vi "GDSIconEditor_HeaderEditorDialog.vi"(0 "NoSplitter":bool, 1 "BodyBackGround":u32(colorbox), 2 "HeaderText":string, 5 "error in (no error)":errorcluster, 6 "HeaderIconIn":u8[][](array[numeric]) format="%x", 7 "Type":T2, 8 "FrameThickness(1)":u32=1, 9 "ClassBodyIcon":string, 10 "FrameColor":u32(colorbox)) -> (14 "NoSplitterOut":bool, 15 "Cancelled":bool, 16 "FrameColorOut":u32(colorbox), 17 "FrameThicknessOut":u32=1, 18 "HeaderIconOut":u8[][](array[numeric]) format="%x", 19 "error out":errorcluster)   [LabVIEW 2020]
uses:
  <resource>/Framework/Providers/Open_GDS/ClassProviders/Common/LvIcon_class/GDSLvIcon_ColorControl.ctl
  <resource>/Framework/Providers/Open_GDS/ClassProviders/Common/LvIcon_class/GDSLvIcon_Type.ctl
  <vilib>/Utility/miscctls.llb/LVPoint32TypeDef.ctl
  <resource>/Framework/Providers/Open_GDS/ClassProviders/Common/LvIcon_class/GDSLvIcon_ClassColorTypes.ctl
  <resource>/Framework/Providers/Open_GDS/ClassProviders/Common/LvIcon_class/subvis/GDSLvIcon_TextDataType.ctl
  <resource>/Framework/Providers/Open_GDS/ClassProviders/Common/LvIcon_class/GDSLvIcon_WordCompressionType.ctl
  <resource>/Framework/Providers/Open_GDS/ClassProviders/Common/LvIcon_class/GDSLvIcon_TextAlignment.ctl
  <vilib>/event_ctls.llb/lveventtype.ctl
  <vilib>/Analysis/NI_AALBase.lvlib
panel:
  out "Coords 2":T1
  out "Coords":T1
  in  "_LastHeaders":picture[](array[picture]) caption="Last used headers"
  in  "Help":bool
  in  "Dice":cluster{"Boolean 2":bool, "Dice 2":bool}
  out "Icon Preview":picture
  in  "Frame":T3 caption="Color"
  in  "Thickness (pixels)":u8=3 min=1 max=3 step=1
  in  "Rows":enum16{"1 Row", "2 Rows", "3 Rows"}(ring)
  in  "Font Compression":enum16{"Auto", "On", "Off"}(ring)
  in  "CapitalOnly":bool=TRUE caption="Only use capital characters"
  in  "Height (pixels)":u8=9 min=5 max=19
  in  "Text":string="Endevo"
  in  "HeaderBk":T3 caption="Background"
  in  "HeaderText":T3 caption="Text"
  in  "OK":bool
  in  "Cancel":bool
  # "Header"
  # "Random color generation"
  # "Frame"
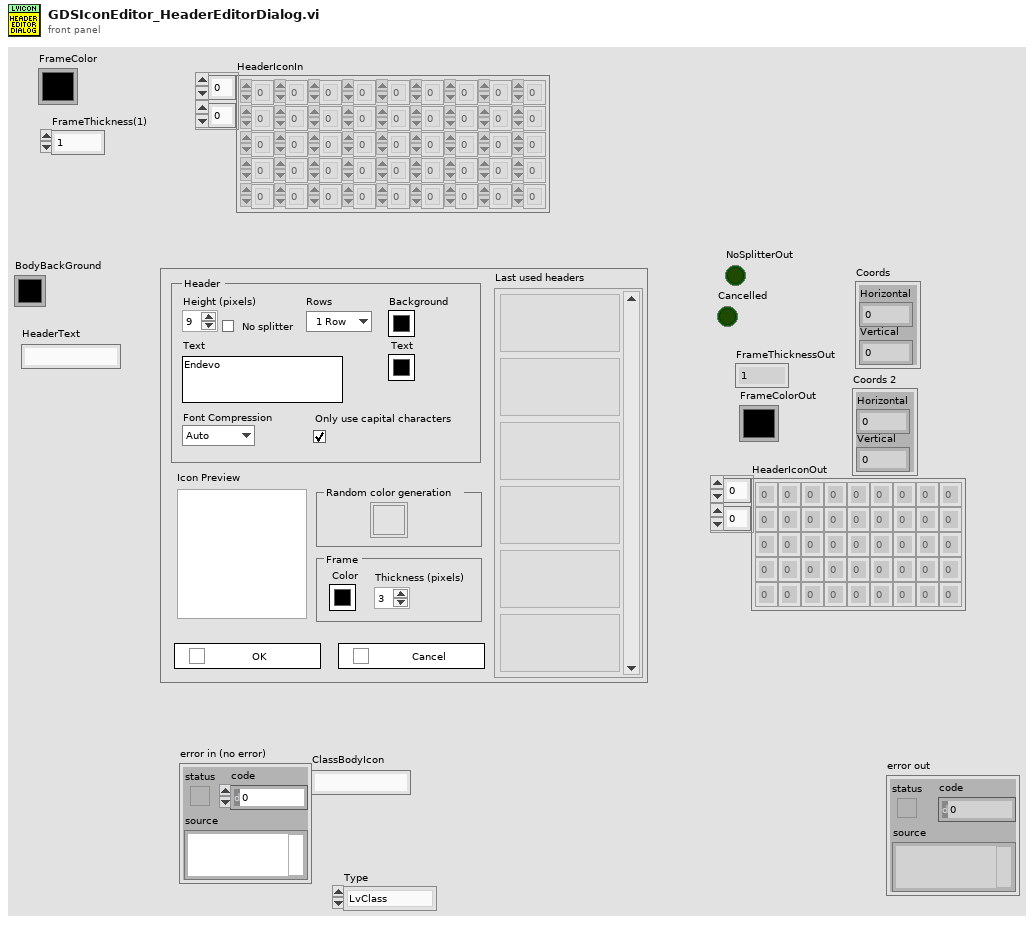
[diagram p1: front panel]
types:
  T1 = typedef "LVPoint32TypeDef.ctl" = cluster{"Horizontal":i32, "Vertical":i32}
  T2 = typedef "GDSLvIcon_Type.ctl" = enum16{"LvClass", "Library", "X-Control", "LvInterface"}
  T3 = typedef "GDSLvIcon_ColorControl.ctl" = cluster{"Decal":bool, "Color":u32}
  T4 = cluster{"Names":string[], "Headers":cluster{"Header":u8[][]}[]}
  T5 = typedef "GDSLvIcon_ClassColorTypes.ctl" = cluster{"Frame":u32, "Header Text Color":u32, "Header Background":u32, "BodyBackgroundPublic":u32, "BodyBackgroundProtected":u32, "BodyBackgroundPrivate":u32, "Body Text Color":u32, "Frame thickness":u8, "ProtectedPrivateSame":bool, "Icon Header Size":u8, "Font Compression":enum16{"Auto", "On", "Off"}, "CapitalOnly":bool}
  T6 = cluster{"Header":u8[][], "Cancel":bool, "Names":string[], "Headers":cluster{"Header":u8[][]}[], "FirstCall":bool}
  T7 = cluster{"Selection Start":u32, "Selection End":u32}
  T8 = cluster{"left":i16, "top":i16, "right":i16, "bottom":i16}
  T9 = typedef "GDSLvIcon_TextDataType.ctl" = cluster{"Text":string, "Allow Only Capital Chars":bool, "Compression":T10, "Alignment":T11}
  T10 = typedef "GDSLvIcon_WordCompressionType.ctl" = enum16{"Auto", "On", "Off"}
  T11 = typedef "GDSLvIcon_TextAlignment.ctl" = enum16{"Center", "Left", "Right"}
  T12 = typedef "lveventtype.ctl" = enum32{"Null", "Timeout", "Annotation Menu Selection", "Annotation Menu Selection?", "App Instance Close", "App Instance Close?", "Autoscale Range Change", "Bookmark Info Change", "Cell Edit", "Cell Edit?", "Cursor Grab", "Cursor Grab?", "Cursor Menu Selection", "Cursor Menu Selection?", "Cursor Move", "Cursor Release", "Data Change", "Direction Change", "Display State Change", "Drag Ended", "Drag Enter", "Drag Leave", "Drag Over", "Drag Source Update", "Drag Starting", "Drag Starting?", "Drop", "Exec State Change", "Key Down", "Key Down?", "Key Repeat", "Key Repeat?", "Key Up", "Listbox Double Click", "Menu Activation?", "Menu Selection (App)", "Menu Selection? (App)", "Menu Selection (User)", "Mouse Down", "Mouse Down?", "Mouse Enter", "Mouse Leave", "Mouse Move", "Mouse Up", "Mouse Wheel", "NI Security User Change (App)", "Pane Size", "Panel Close", "Panel Close?", "Panel Resize", "Plot Attribute Change", "Scale Range Change", "Shortcut Menu Activation?", "Shortcut Menu Selection (App)", "Shortcut Menu Selection? (App)", "Shortcut Menu Selection (User)", "Tree Double Click", "Tree Drag", "Tree Drag?", "Tree Drop", "Tree Drop?", "Tree Item Close", "Tree Item Close?", "Tree Item Open", "Tree Item Open?", "User Event", "Value Change"}
  T13 = typedef "ColorControl.ctl" = cluster{"Decal":bool, "Color":u32}
  T14 = typedef "LVRectTypeDef.ctl" = cluster{"Left":i16, "Top":i16, "Right":i16, "Bottom":i16}
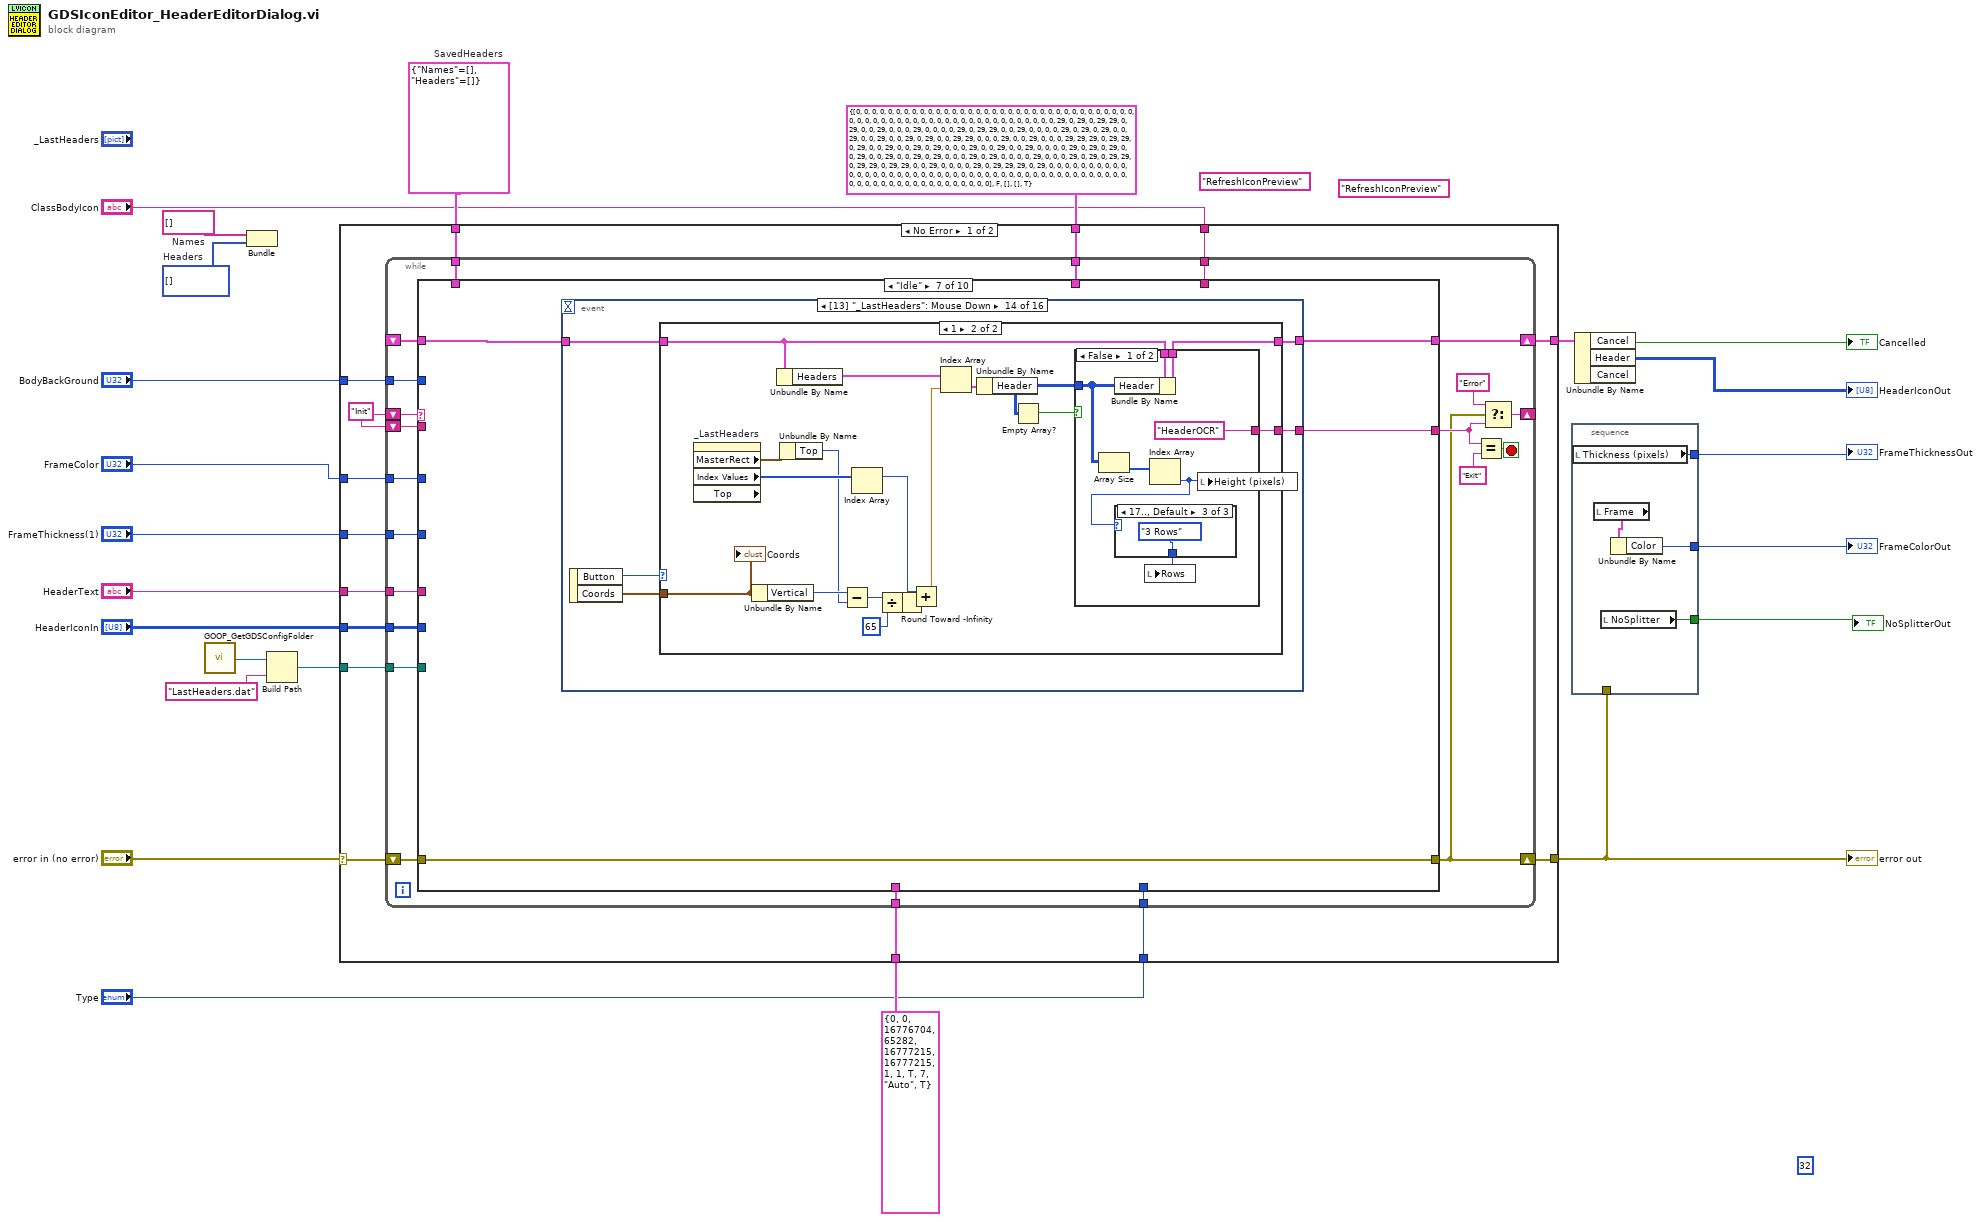
[diagram p0: block diagram]
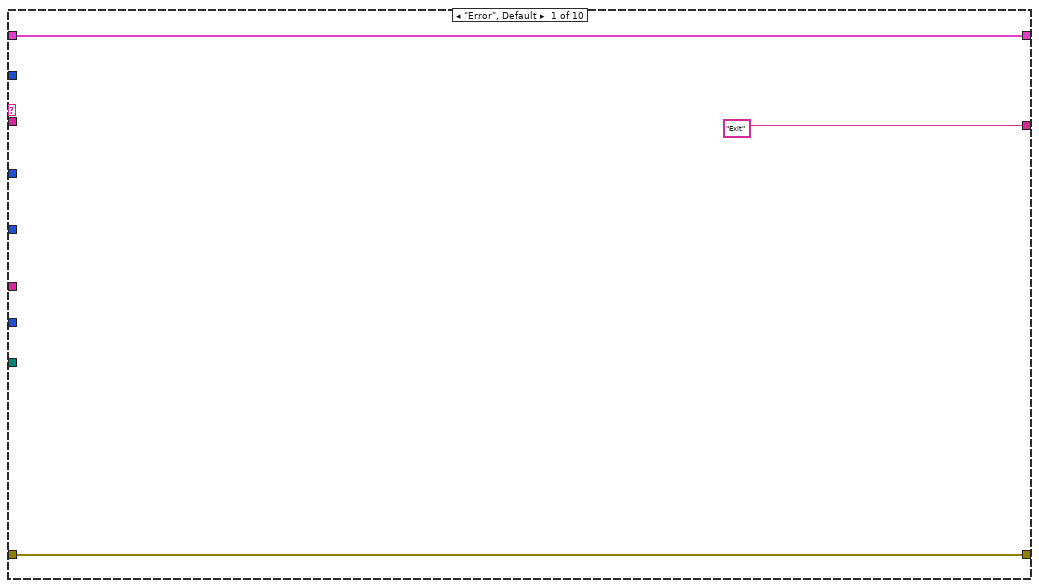
[diagram p2: hidden frame]
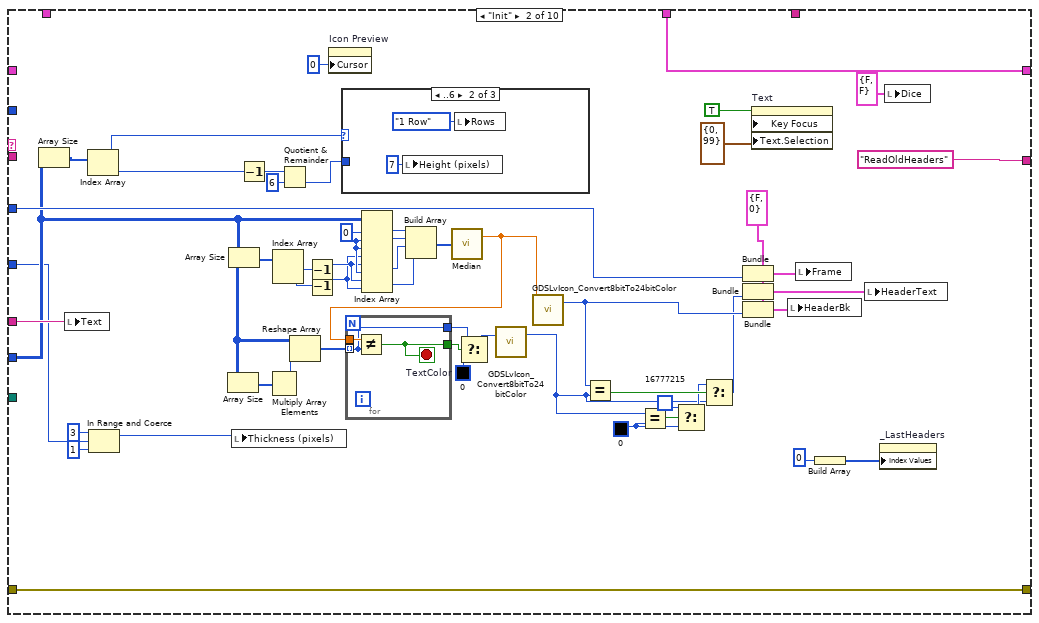
[diagram p3: hidden frame]
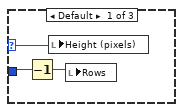
[diagram p4: hidden frame]
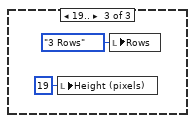
[diagram p5: hidden frame]
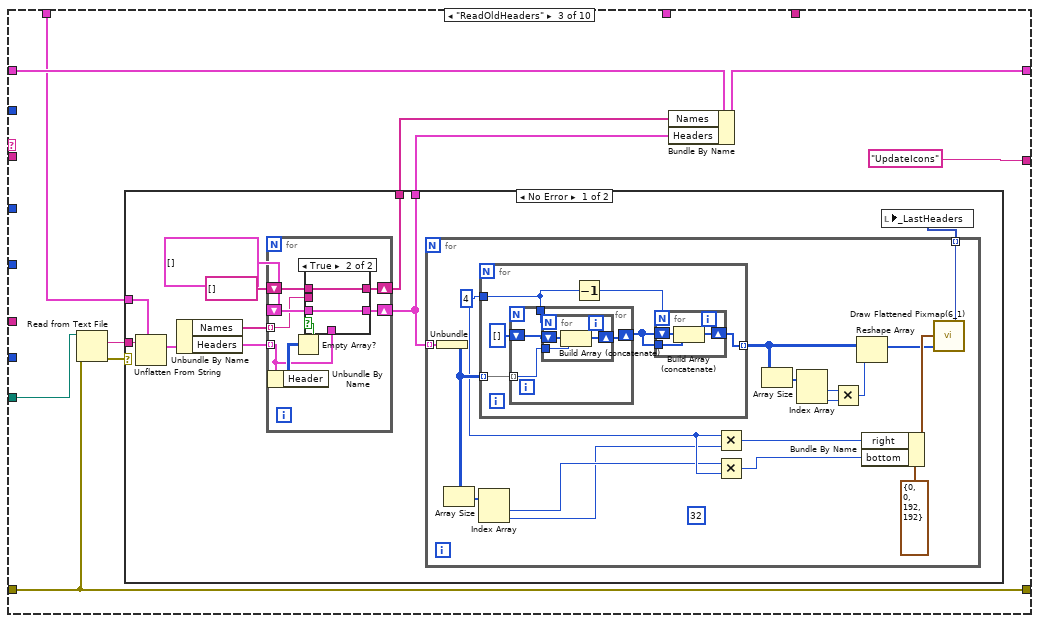
[diagram p6: hidden frame]
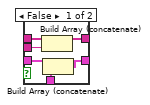
[diagram p7: hidden frame]
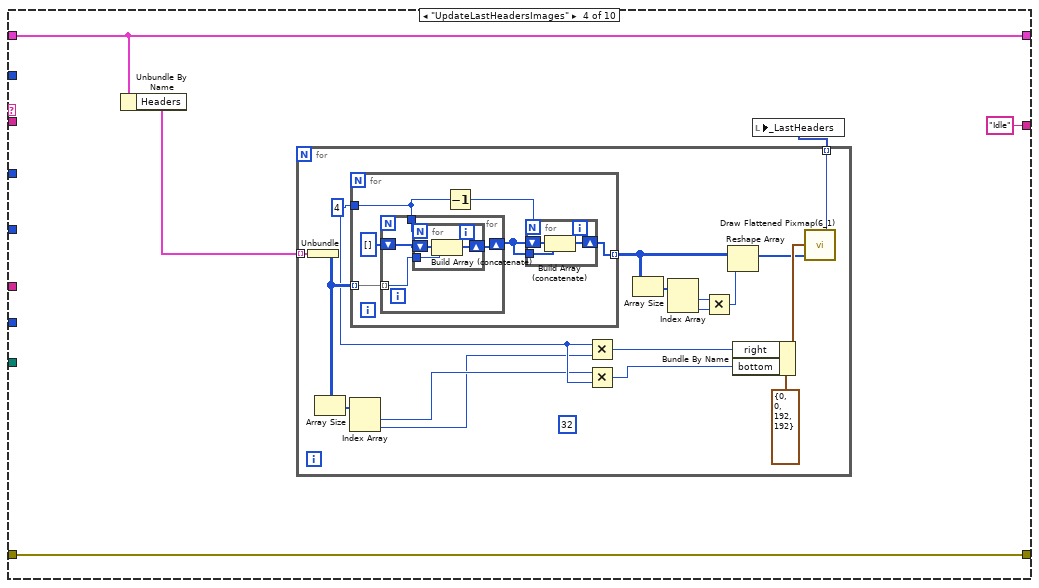
[diagram p9: hidden frame]
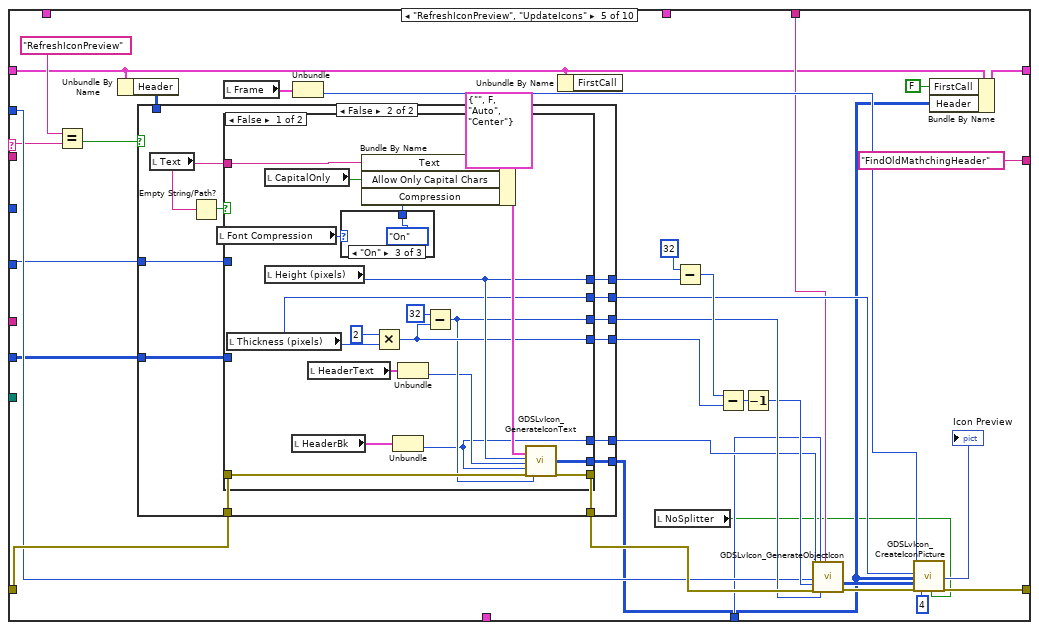
[diagram p10: hidden frame]
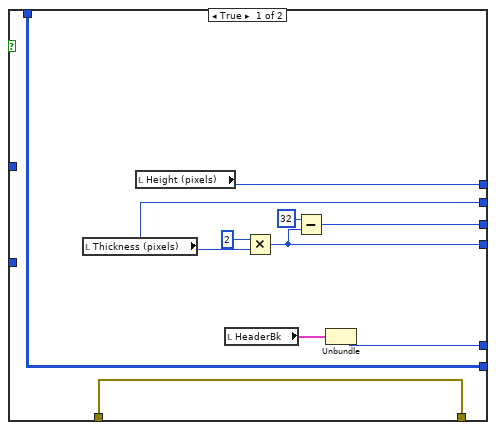
[diagram p11: hidden frame]
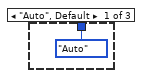
[diagram p12: hidden frame]
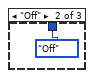
[diagram p13: hidden frame]
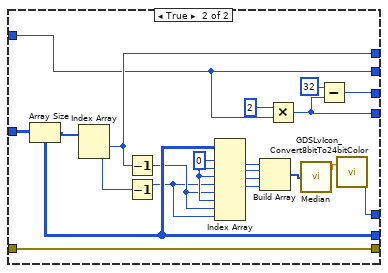
[diagram p14: hidden frame]
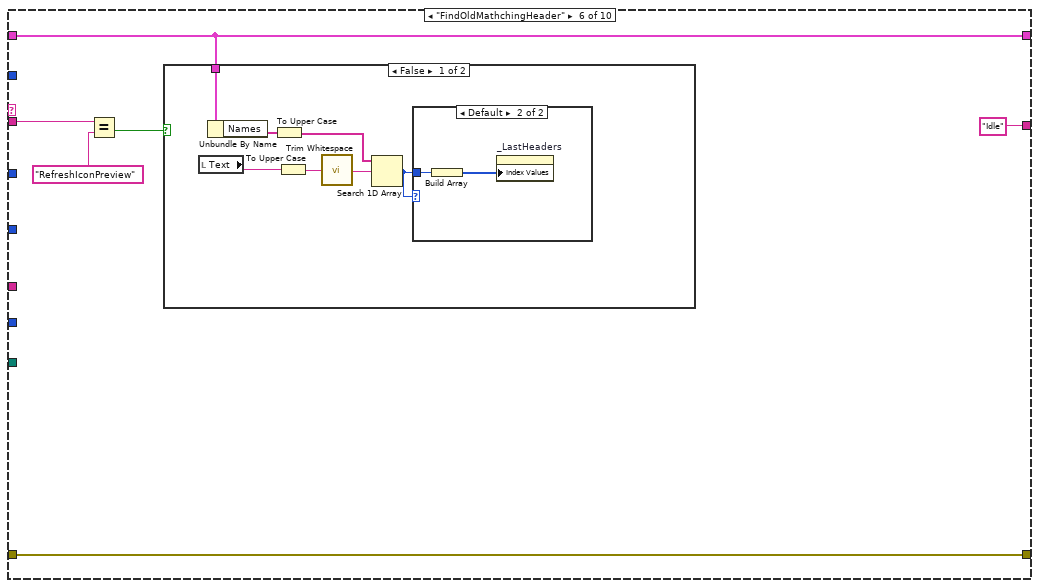
[diagram p15: hidden frame]
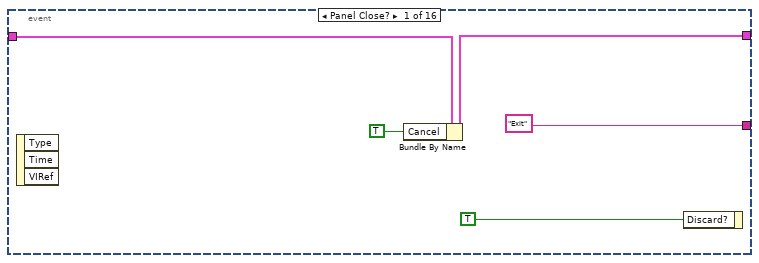
[diagram p18: hidden frame]
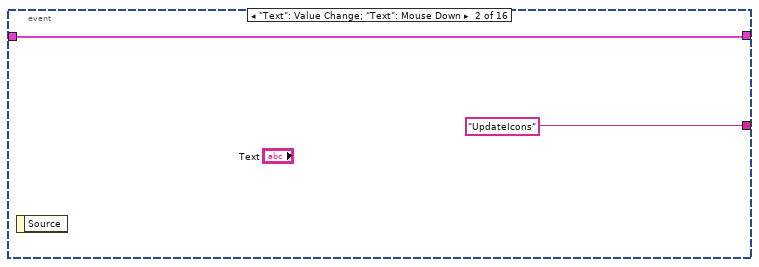
[diagram p19: hidden frame]
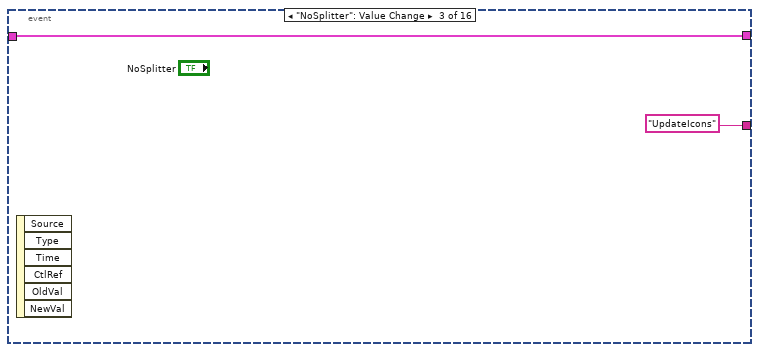
[diagram p20: hidden frame]
diagram:
  (unwired) "RefreshIconPreview"
  (unwired) "RefreshIconPreview"
  w3 = T4 {"Names"=[], "Headers"=[]}  # SavedHeaders
  (unwired) i16 32 ("bottom")
  w5 = picture[] []  # Headers
  w4 = string[] []  # Names
  n1 = call <resource>:"GOOP_GetGDSConfigFolder.vi"() -> ("GDSFolderPath"=w7:path)
  n2 = Bundle("Names"=w4, "Headers"=w5) -> ()  [unwired: 1 in, 1 out]
  n3 = Build Path(base path=w7, name or relative path="LastHeaders.dat") -> (appended path=w6:path)
  n4 = case shown="No Error" "error in (no error)" {
    selector: "error in (no error)" -> [w38 w580]
    tunnel: [w37 w580] -> w13
    tunnel: "BodyBackGround" -> [w36 _]
    tunnel: T6 {"Header"=[[0, 0, 0, 0, 0, 0, 0, 0, 0, 0, 0, 0, 0, 0, 0, 0, 0, 0, 0, 0, 0, 0, 0, 0, 0, 0, 0, 0, 0, 0], [0, 0, 0, 0, 0, 0, 0, 0, 0, 0, 0, 0, 0, 0, 0, 0, 0, 0, 0, 0, 0, 0, 0, 0, 0, 0, 0, 0, 0, 0], [0, 29, 0, 29, 0, 29, 29, 0, 29, 0, 0, 29, 0, 0, 0, 29, 0, 0, 0, 0, 29, 0, 29, 29, 0, 0, 29, 0, 0, 0], [0, 29, 0, 29, 0, 29, 0, 0, 29, 0, 0, 29, 0, 0, 29, 0, 29, 0, 0, 29, 29, 0, 0, 0, 29, 0, 0, 29, 0, 0], [0, 29, 29, 29, 0, 29, 29, 0, 29, 0, 0, 29, 0, 0, 29, 0, 29, 0, 0, 0, 29, 0, 0, 29, 0, 0, 29, 0, 0, 0], [0, 29, 0, 29, 0, 29, 0, 0, 29, 0, 0, 29, 0, 0, 29, 0, 29, 0, 0, 0, 29, 0, 29, 0, 0, 0, 0, 29, 0, 0], [0, 29, 0, 29, 0, 29, 29, 0, 29, 29, 0, 29, 29, 0, 0, 29, 0, 0, 0, 0, 29, 0, 29, 29, 29, 0, 29, 0, 0, 0], [0, 0, 0, 0, 0, 0, 0, 0, 0, 0, 0, 0, 0, 0, 0, 0, 0, 0, 0, 0, 0, 0, 0, 0, 0, 0, 0, 0, 0, 0], [0, 0, 0, 0, 0, 0, 0, 0, 0, 0, 0, 0, 0, 0, 0, 0, 0, 0, 0, 0, 0, 0, 0, 0, 0, 0, 0, 0, 0, 0]], "Cancel"=FALSE, "Names"=[], "Headers"=[], "FirstCall"=TRUE} -> [w35 _]
    tunnel: T5 {"Frame"=0, "Header Text Color"=0, "Header Background"=16776704, "BodyBackgroundPublic"=65282, "BodyBackgroundProtected"=16777215, "BodyBackgroundPrivate"=16777215, "Body Text Color"=1, "Frame thickness"=1, "ProtectedPrivateSame"=TRUE, "Icon Header Size"=7, "Font Compression"=enum."Auto", "CapitalOnly"=TRUE} ("type") -> [w34 _]
    tunnel: "FrameThickness(1)" -> [w33 _]
    tunnel: "FrameColor" -> [w32 _]
    tunnel: "HeaderText" -> [w31 _]
    tunnel: [w30 _] -> w16
    tunnel: "HeaderIconIn" -> [w29 _]
    tunnel: "Type" -> [w28 _]
    tunnel: w6 -> [w27 _]
    tunnel: w3 -> [w26 _]
    tunnel: "ClassBodyIcon" -> [w24 _]
    frame No Error {
      w25 = "Init"
      n5 = while {
        shift-right: [w53] -> w37
        shift-left: w38 -> [w60]
        shift-right: [w58] -> _
        shift-left: w25 -> [w59]
        shift-right: [w42] -> w30
        shift-left: _ -> [w52]
        tunnel: w36 -> [w51]
        tunnel: w35 -> [w50]
        tunnel: w34 -> [w49]
        tunnel: w33 -> [w48]
        tunnel: w32 -> [w47]
        tunnel: w31 -> [w46]
        tunnel: w29 -> [w45]
        tunnel: w28 -> [w44]
        tunnel: w27 -> [w43]
        tunnel: w26 -> [w41]
        shift-left: w25 -> [w40]
        tunnel: w24 -> [w39]
        stop <- w57 stop-if-true
        n6 = case shown="\"Idle\"" w59 {
          selector: w59 -> [_ _ _ _ w241 _ _ _ _ _]
          tunnel: w60 -> [w63 w106 w128 w198 w265 w333 w347 w462 w520 w537]
          tunnel: [w63 w106 w128 w198 w257 w333 w347 w462 w520 w537] -> w53
          tunnel: ["Exit" "ReadOldHeaders" "UpdateIcons" "Idle" "FindOldMathchingHeader" "Idle" w348 "RefreshIconPreview" "UpdateIcons" "Exit"] -> w54
          tunnel: w52 -> [w61 _ w131 w196 w235 w334 w346 w494 w535 w545]
          tunnel: w51 -> [_ _ _ _ w245 _ _ _ _ _]
          tunnel: w50 -> [_ w105 _ _ _ _ _ _ _ _]
          tunnel: w49 -> [_ _ _ _ _ _ _ _ _ _]
          tunnel: w48 -> [_ w70 _ _ w243 _ _ _ _ _]
          tunnel: w47 -> [_ w109 _ _ _ _ _ _ _ _]
          tunnel: w46 -> [_ w104 _ _ _ _ _ _ _ _]
          tunnel: w45 -> [_ w76 _ _ w244 _ _ _ _ _]
          tunnel: w44 -> [_ _ _ _ w242 _ _ _ _ _]
          tunnel: w43 -> [_ _ w134 _ _ _ _ _ _ w539]
          tunnel: [w61 w105 w130 w196 w251 w334 w345 w494 w535 w545] -> w42
          tunnel: w41 -> [_ _ w126 _ _ _ _ _ _ w540]
          tunnel: w40 -> [_ _ _ _ _ w332 _ _ _ _]
          tunnel: w39 -> [_ _ _ _ w238 _ _ _ _ _]
          frame "Error", Default {
          }
          frame "Init" {
            w110 = T3 {"Decal"=FALSE, "Color"=0} ("Frame")
            w77 = u32 0  # TextColor
            w91 = 0 ("index (row)")
            w71 = u32 0
            n7 = Array Size(array=w76) -> (size(s)=w103:i32[])
            n8 = local write "Text"(w104) -> ()
            n9 = Index Array(array=w103) -> (element=w100:i32)  [unwired: 1 in]
            n10 = In Range and Coerce(upper limit=u32 3, x=w70, lower limit=u32 1) -> (coerced(x)=w67:u32)  [unwired: 1 out]
            n11 = Array Size(array=w76) -> (size(s)=w83:i32[])
            n12 = Array Size(array=w76) -> (size(s)=w94:i32[])
            n13 = local write "Thickness (pixels)"(w67) -> ()
            n14 = Decrement(x=w100) -> (x-1=w102:i32)
            n15 = Multiply Array Elements(1:w83) -> (0:w81:i32)
            n16 = Index Array(array=w94) -> (element #1=w93:i32, element #2=w92:i32)  [unwired: 2 in]
            n17 = Quotient & Remainder(x=w102, y=6) -> (floor(x/y)=w99:i32)  [unwired: 1 out]
            n18 = Reshape Array(w76, w81) -> (w82:u8[])
            n19 = Decrement(x=w93) -> (x-1=w90:i32)
            n20 = Decrement(x=w92) -> (x-1=w89:i32)
            n21 = property on="Icon Preview" class="Pict"("Cursor"=0) -> ()  [unwired: 2 in, 2 out]
            n22 = case shown="..6" w100 {
              selector: w100 -> [w121 _ _]
              tunnel: w99 -> [w120 _ _]
              frame Default {
                n23 = Decrement(x=w120) -> (x-1=w119:i32)
                n24 = local write "Height (pixels)"(w121) -> ()
                n25 = local write "Rows"(w119) -> ()
              }
              frame ..6 {
                n26 = local write "Height (pixels)"(u8 7 ("Height (pixels)")) -> ()
                n27 = local write "Rows"(enum16{"1 Row", "2 Rows", "3 Rows"}."1 Row" ("Rows")) -> ()
              }
              frame 19.. {
                n28 = local write "Height (pixels)"(u8 19 ("Height (pixels)")) -> ()
                n29 = local write "Rows"(enum16{"1 Row", "2 Rows", "3 Rows"}."3 Rows" ("Rows")) -> ()
              }
            }
            n30 = Index Array(array=w76, index (row) #1=w91, index (col) #1=w91, index (row) #2=w91, index (col) #2=w89, index (row) #3=w90, index (col) #3=w91, index (row) #4=w90, index (col) #4=w89) -> (element #1=w88:u8, element #2=w87:u8, element #3=w86:u8, element #4=w85:u8)
            n31 = Build Array(w88, w87, w86, w85) -> (w84:u8[])
            n32 = call <vilib>:"Median.vi"("X"=w84) -> ("median"=w75:dbl)  [unwired: 1 out]
            n33 = for {
              tunnel: w82 -> [w117] mode=indexing
              tunnel: w75 -> [w118]
              tunnel: [w116] -> w79
              tunnel: [w117] -> w78
              stop <- w116 stop-if-true
              n34 = Not Equal?(x=w118, y=w117) -> (x != y?=w116:bool)
            }
            n35 = Select(t=w78, s=w79, f=w77) -> (s? t:f=w80:u32)
            n36 = call <resource>:"GDSLvIcon_Convert8bitTo24bitColor.vi"("Color8bit"=w80) -> ("Color24bit"=w72:u32)  [unwired: 17 in, 1 out]
            n37 = call <resource>:"GDSLvIcon_Convert8bitTo24bitColor.vi"("Color8bit"=w75) -> ("Color24bit"=w74:u32)  [unwired: 17 in, 1 out]
            n38 = Equal?(x=w74, y=w72) -> (x = y?=w98:bool)
            n39 = Equal?(x=w72, y=w71) -> (x = y?=w97:bool)
            n40 = Select(t=u32 16777215, s=w97, f=w71) -> (s? t:f=w95:u32)
            n41 = Select(t=w95, s=w98, f=w72) -> (s? t:f=w73:u32)
            n42 = Bundle(cluster=w110, "Color"=w109) -> (w113:T3)  [unwired: 1 in]
            n43 = Bundle(cluster=w110, "Color"=w73) -> (w112:T3)  [unwired: 1 in]
            n44 = Bundle(cluster=w110, "Color"=w74) -> (w111:T3)  [unwired: 1 in]
            n45 = property on="Text" class="Str"("Key Focus"=TRUE, "Text.Selection"=T7 {"Selection Start"=0, "Selection End"=99}) -> ()  [unwired: 2 in, 2 out]
            n46 = local write "HeaderBk"(w111) -> ()
            n47 = local write "Frame"(w113) -> ()
            n48 = Build Array(u32 0) -> (w66:u32[])
            n49 = local write "HeaderText"(w112) -> ()
            n50 = property on="_LastHeaders" class="Arr (strict)"("Index Values"=w66) -> ()  [unwired: 2 in, 2 out]
            n51 = local write "Dice"(cluster{"Boolean 2":bool, "Dice":bool} {"Boolean 2"=FALSE, "Dice"=FALSE} ("Dice")) -> ()
          }
          frame "ReadOldHeaders" {
            n52 = Read from Text File(file (use dialog)=w134, error in=w128) -> (text=w132:string, error out=w133:errorcluster)  [unwired: 2 in, 2 out]
            n53 = case shown="No Error" w133 {
              tunnel: w132 -> [w145 _]
              tunnel: w126 -> [w144 _]
              tunnel: [w136 _] -> w129
              tunnel: [w137 _] -> w127
              frame No Error {
                n54 = Unflatten From String(type=w144, binary string=w145) -> (value=w143:T4)  [unwired: 3 in, 2 out]
                n55 = Unbundle By Name(w143) -> ("Names"=w141:string[], "Headers"=w140:cluster{"Header":u8[][]}[])
                n56 = for {
                  tunnel: w141 -> [w148] mode=indexing
                  tunnel: w140 -> [w146] mode=indexing
                  shift-right: [w149] -> w136
                  shift-left: string[] [] -> [w151]
                  shift-right: [w147] -> w137
                  shift-left: cluster{"Header":u8[][]}[] [] -> [w150]
                  n57 = Unbundle By Name(w146) -> ("Header"=w153:u8[][])
                  n58 = Empty Array?(array=w153) -> (empty?=w152:bool)
                  n59 = case shown="True" w152 {
                    tunnel: w151 -> [w158 w160]
                    tunnel: w150 -> [w156 w161]
                    tunnel: [w159 w160] -> w149
                    tunnel: w148 -> [w157 _]
                    tunnel: [w155 w161] -> w147
                    tunnel: w146 -> [w154 _]
                    frame False {
                      n60 = Build Array (concatenate)(w158, w157) -> (w159:string[])
                      n61 = Build Array (concatenate)(w156, w154) -> (w155:cluster{"Header":u8[][]}[])
                    }
                    frame True {
                    }
                  }
                }
                n62 = for {
                  tunnel: w137 -> [w178] mode=indexing
                  tunnel: [w168] -> w142 mode=indexing
                  w165 = 4 ("BigSizeIcon(x6)")
                  (unwired) 32 ("y")
                  n63 = Unbundle(w178) -> ("Header"=w166:u8[][])
                  n64 = Array Size(array=w166) -> (size(s)=w167:i32[])
                  n65 = Index Array(array=w167) -> (element #1=w163:i32, element #2=w162:i32)  [unwired: 2 in]
                  n66 = for {
                    tunnel: w166 -> [w184] mode=indexing
                    tunnel: [w182] -> w173 mode=indexing
                    tunnel: w165 -> [w179]
                    n67 = for {
                      tunnel: w184 -> [w191] mode=indexing
                      shift-right: [w189] -> w181
                      shift-left: u8[] [] -> [w190]
                      tunnel: w179 -> [w188]
                      n68 = for {
                        N: w188 -> [_]
                        tunnel: w191 -> [w194]
                        shift-right: [w192] -> w189
                        shift-left: w190 -> [w193]
                        n69 = Build Array (concatenate)(w193, w194) -> (w192:u8[])
                      }
                    }
                    n70 = Decrement(x=w179) -> (x-1=w180:i32)
                    n71 = for {
                      N: w180 -> [_]
                      tunnel: w181 -> [w187]
                      shift-right: [w185] -> w182
                      shift-left: w181 -> [w186]
                      n72 = Build Array (concatenate)(w186, w187) -> (w185:u8[])
                    }
                  }
                  n73 = Multiply(x=w165, y=w162) -> (x*y=w177:i32)
                  n74 = Multiply(x=w163, y=w165) -> (x*y=w164:i32)
                  n75 = Array Size(array=w173) -> (size(s)=w169:i32[])
                  n76 = Index Array(array=w169) -> (element #1=w171:i32, element #2=w170:i32)  [unwired: 2 in]
                  n77 = Multiply(x=w171, y=w170) -> (x*y=w172:i32)
                  n78 = Reshape Array(w173, w172) -> (w174:u8[])
                  n79 = Bundle By Name(cluster=T8 {"left"=0, "top"=0, "right"=192, "bottom"=192} ("rect"), "right"=w177, "bottom"=w164) -> (w176:T8)
                  n80 = call <vilib>:"Draw Flattened Pixmap(6_1).vi"("rect"=w176, "flattened pixmap data"=w174) -> ("new picture"=w168:picture)  [unwired: 7 in]
                }
                n81 = local write "_LastHeaders"(w142) -> ()
              }
              frame Error {
              }
            }
            n82 = Bundle By Name(cluster=w131, "Names"=w129, "Headers"=w127) -> (w130:T6)
          }
          frame "UpdateLastHeadersImages" {
            n83 = Unbundle By Name(w196) -> ("Headers"=w197:cluster{"Header":u8[][]}[])
            n84 = for {
              tunnel: w197 -> [w216] mode=indexing
              tunnel: [w206] -> w199 mode=indexing
              w203 = 4 ("BigSizeIcon(x6)")
              (unwired) 32 ("y")
              n85 = Unbundle(w216) -> ("Header"=w204:u8[][])
              n86 = Array Size(array=w204) -> (size(s)=w205:i32[])
              n87 = Index Array(array=w205) -> (element #1=w201:i32, element #2=w200:i32)  [unwired: 2 in]
              n88 = for {
                tunnel: w204 -> [w222] mode=indexing
                tunnel: [w220] -> w211 mode=indexing
                tunnel: w203 -> [w217]
                n89 = for {
                  tunnel: w222 -> [w229] mode=indexing
                  shift-right: [w227] -> w219
                  shift-left: u8[] [] -> [w228]
                  tunnel: w217 -> [w226]
                  n90 = for {
                    N: w226 -> [_]
                    tunnel: w229 -> [w232]
                    shift-right: [w230] -> w227
                    shift-left: w228 -> [w231]
                    n91 = Build Array (concatenate)(w231, w232) -> (w230:u8[])
                  }
                }
                n92 = Decrement(x=w217) -> (x-1=w218:i32)
                n93 = for {
                  N: w218 -> [_]
                  tunnel: w219 -> [w225]
                  shift-right: [w223] -> w220
                  shift-left: w219 -> [w224]
                  n94 = Build Array (concatenate)(w224, w225) -> (w223:u8[])
                }
              }
              n95 = Multiply(x=w203, y=w200) -> (x*y=w215:i32)
              n96 = Multiply(x=w201, y=w203) -> (x*y=w202:i32)
              n97 = Array Size(array=w211) -> (size(s)=w207:i32[])
              n98 = Index Array(array=w207) -> (element #1=w209:i32, element #2=w208:i32)  [unwired: 2 in]
              n99 = Multiply(x=w209, y=w208) -> (x*y=w210:i32)
              n100 = Reshape Array(w211, w210) -> (w212:u8[])
              n101 = Bundle By Name(cluster=T8 {"left"=0, "top"=0, "right"=192, "bottom"=192} ("rect"), "right"=w215, "bottom"=w202) -> (w214:T8)
              n102 = call <vilib>:"Draw Flattened Pixmap(6_1).vi"("rect"=w214, "flattened pixmap data"=w212) -> ("new picture"=w206:picture)  [unwired: 7 in]
            }
            n103 = local write "_LastHeaders"(w199) -> ()
          }
          frame "RefreshIconPreview", "UpdateIcons" {
            n104 = Equal?(x="RefreshIconPreview", y=w241) -> (x = y?=w237:bool)
            n105 = Unbundle By Name(w235) -> ("Header"=w239:u8[][])
            n106 = case shown="False" w237 {
              tunnel: w265 -> [w269 w287]
              tunnel: [w269 w286] -> w263
              tunnel: [w275 w285] -> w259
              tunnel: [w274 w284] -> w255
              tunnel: [w273 w283] -> w254
              tunnel: [w272 w282] -> w253
              tunnel: [w268 w281] -> w236
              tunnel: [w266 w280] -> w247
              tunnel: w244 -> [_ w277]
              tunnel: w243 -> [_ w276]
              tunnel: w239 -> [w268 _]
              frame True {
                n107 = local read "Thickness (pixels)"() -> (w273:u8)
                n108 = local read "Height (pixels)"() -> (w275:u8)
                n109 = local read "HeaderBk"() -> (w267:T3)
                n110 = Multiply(x=u8 2, y=w273) -> (x*y=w274:u8)
                n111 = Subtract(x=32, y=w274) -> (x-y=w272:i32)
                n112 = Unbundle(w267) -> ("Color"=w266:u32)  [unwired: 1 out]
              }
              frame False {
                n113 = local read "Text"() -> (w278:string)
                n114 = Empty String/Path?(string/path=w278) -> (empty?=w279:bool)
                n115 = case shown="False" w279 {
                  tunnel: w287 -> [w306 w329]
                  tunnel: [w301 w329] -> w286
                  tunnel: [w299 w323] -> w285
                  tunnel: [w297 w324] -> w284
                  tunnel: [w295 w312] -> w283
                  tunnel: [w294 w325] -> w282
                  tunnel: [w293 w321] -> w281
                  tunnel: [w289 w310] -> w280
                  tunnel: w278 -> [w288 _]
                  tunnel: w277 -> [_ w321]
                  tunnel: w276 -> [_ w312]
                  frame False {
                    n116 = local read "Font Compression"() -> (w304:enum16{"Auto", "On", "Off"})
                    n117 = local read "Thickness (pixels)"() -> (w295:u8)
                    n118 = local read "CapitalOnly"() -> (w296:bool)
                    n119 = local read "Height (pixels)"() -> (w299:u8)
                    n120 = local read "HeaderBk"() -> (w290:T3)
                    n121 = local read "HeaderText"() -> (w292:T3)
                    n122 = case shown="\"On\"" w304 {
                      tunnel: [enum16{"Auto", "On", "Off"}."Auto" ("Compression") enum16{"Auto", "On", "Off"}."Off" ("Compression") enum16{"Auto", "On", "Off"}."On" ("Compression")] -> w305
                      frame "Auto", Default {
                      }
                      frame "Off" {
                      }
                      frame "On" {
                      }
                    }
                    n123 = Bundle By Name(cluster=T9 {"Text"="", "Allow Only Capital Chars"=FALSE, "Compression"=enum."Auto", "Alignment"=enum."Center"} ("Text"), "Text"=w288, "Allow Only Capital Chars"=w296, "Compression"=w305) -> (w302:T9)
                    n124 = Multiply(x=u8 2, y=w295) -> (x*y=w297:u8)
                    n125 = Unbundle(w290) -> ("Color"=w289:u32)  [unwired: 1 out]
                    n126 = Unbundle(w292) -> ("Color"=w291:u32)  [unwired: 1 out]
                    n127 = Subtract(x=32, y=w297) -> (x-y=w294:i32)
                    n128 = call <resource>:"GDSLvIcon_GenerateIconText.vi"("Text"=w302, "TextPixelHeight(5-30)"=w299, "Foreground color"=w291, "Background color"=w289, "error in (no error)"=w306, "Text Pixel width(32-FrameThicknes*2))"=w294) -> ("TextOut"=w293:u8[][], "error out"=w301:errorcluster)  [unwired: 9 in, 3 out]
                  }
                  frame True {
                    w320 = 0 ("index (row)")
                    n129 = Array Size(array=w321) -> (size(s)=w328:i32[])
                    n130 = Index Array(array=w328) -> (element #1=w323:i32, element #2=w322:i32)  [unwired: 2 in]
                    n131 = Decrement(x=w323) -> (x-1=w319:i32)
                    n132 = Decrement(x=w322) -> (x-1=w318:i32)
                    n133 = Index Array(array=w321, index (row) #1=w320, index (col) #1=w320, index (row) #2=w320, index (col) #2=w318, index (row) #3=w319, index (col) #3=w320, index (row) #4=w319, index (col) #4=w318) -> (element #1=w317:u8, element #2=w316:u8, element #3=w315:u8, element #4=w314:u8)
                    n134 = Build Array(w317, w316, w315, w314) -> (w313:u8[])
                    n135 = Multiply(x=u8 2, y=w312) -> (x*y=w324:u32)
                    n136 = call <vilib>:"Median.vi"("X"=w313) -> ("median"=w311:dbl)  [unwired: 1 out]
                    n137 = Subtract(x=32, y=w324) -> (x-y=w325:u32)
                    n138 = call <resource>:"GDSLvIcon_Convert8bitTo24bitColor.vi"("Color8bit"=w311) -> ("Color24bit"=w310:u32)  [unwired: 17 in, 1 out]
                  }
                }
              }
            }
            n139 = local read "Frame"() -> (w248:T3)
            n140 = Unbundle(w248) -> ("Color"=w249:u32)  [unwired: 1 out]
            n141 = Unbundle By Name(w235) -> ()  [unwired: 1 out]
            n142 = local read "NoSplitter"() -> (w233:bool)
            n143 = Subtract(x=32, y=w259) -> (x-y=w262:i32)
            n144 = Subtract(x=w262, y=w255) -> (x-y=w261:u32)
            n145 = Decrement(x=w261) -> (x-1=w252:u32)
            n146 = call <resource>:"GDSLvIcon_GenerateObjectIcon.vi"("HeaderColor"=w247, "BackgroundColor"=w245, "Height"=w252, "error in (no error)"=w263, "Type"=w242, "Width(30)"=w253, "ClassBodyIcon"=w238) -> ("BodyIconOut"=w250:u8[][], "error out"=w258:errorcluster)  [unwired: 11 in]
            n147 = call <resource>:"GDSLvIcon_CreateIconPicture.vi"("FrameColor"=w249, "FrameThickness(1)"=w254, "HeaderIconIn"=w236, "BodyIconIn"=w250, "error in (no error)"=w258, "BigSizeIcon(x6)"=4, "0px Splitter(False)"=w233) -> ("LargeIconPictureOut(x6)"=→"Icon Preview":picture, "error out"=w257:errorcluster)  [unwired: 7 in, 4 out]
            n148 = Bundle By Name(cluster=w235, "FirstCall"=FALSE, "Header"=w236) -> (w251:T6)
          }
          frame "FindOldMathchingHeader" {
            n149 = Equal?(x=w332, y="RefreshIconPreview") -> (x = y?=w330:bool)
            n150 = case shown="False" w330 {
              tunnel: w334 -> [w342 _]
              frame False {
                n151 = local read "Text"() -> (w340:string)
                n152 = Unbundle By Name(w342) -> ("Names"=w341:string[])
                n153 = To Upper Case(1:w341) -> (0:w337:string[])
                n154 = To Upper Case(1:w340) -> (0:w339:string)
                n155 = call <vilib>:"Trim Whitespace.vi"("string"=w339) -> ("trimmed string"=w338:string)  [unwired: 1 in]
                n156 = Search 1D Array(1D array=w337, element=w338) -> (index of element=w336:i32)  [unwired: 1 in]
                n157 = case shown="Default" w336 {
                  tunnel: w336 -> [_ w344]
                  frame -1 {
                  }
                  frame Default {
                    n158 = Build Array(w344) -> (w343:i32[])
                    n159 = property on="_LastHeaders" class="Arr (strict)"("Index Values"=w343) -> ()  [unwired: 2 in, 2 out]
                  }
                }
              }
              frame True {
              }
            }
          }
          frame "Idle" {
            n160 = event shown="[13] \"_LastHeaders\": Mouse Down" {
              selector: _ -> [_ _ _ _ _ _ _ _ _ _ _ _ _ _ _ _]
              dyn-events: _ -> [_ _ _ _ _ _ _ _ _ _ _ _ _ _ _ _]
              timeout: _ -> [_ _ _ _ _ _ _ _ _ _ _ _ _ _ _ _]
              tunnel: ["Exit" "UpdateIcons" "UpdateIcons" "Idle" "Idle" "Idle" "RandomColors" "UpdateIcons" "Idle" "UpdateIcons" "RefreshIconPreview" "RefreshIconPreview" "UpdateLastHeaders" w403 "UpdateLastHeadersImages" "Exit"] -> w348
              tunnel: w346 -> [w351 w354 w357 w360 w362 w365 w367 w369 w372 w380 w388 w390 w398 w401 w441 w456]
              tunnel: [w349 w354 w357 w360 w362 w365 w367 w369 w372 w380 w388 w390 w398 w402 w440 w455] -> w345
              event Panel Close? {
                n161 = event-data() -> ()  [unwired: 1 in, 3 out]
                n162 = Bundle By Name(cluster=w351, "Cancel"=TRUE) -> (w349:T6)
                n163 = event-data("Discard?"=TRUE) -> ()  [unwired: 1 in, 1 out]
              }
              event "Text": Value Change; "Text": Mouse Down {
                n164 = event-data() -> ()  [unwired: 1 in, 1 out]
              }
              event "NoSplitter": Value Change {
                n165 = event-data() -> ()  [unwired: 1 in, 6 out]
              }
              event "Dice": Mouse Enter {
                n166 = event-data() -> ()  [unwired: 1 in, 1 out]
                n167 = local write "Dice"(cluster{"Boolean 2":bool, "Dice":bool} {"Boolean 2"=TRUE, "Dice"=FALSE} ("Dice")) -> ()
              }
              event "Help": Value Change {
                n168 = event-data() -> ()  [unwired: 1 in, 6 out]
              }
              event "Dice": Mouse Leave {
                n169 = event-data() -> ()  [unwired: 1 in, 1 out]
                n170 = local write "Dice"(cluster{"Boolean 2":bool, "Dice":bool} {"Boolean 2"=FALSE, "Dice"=FALSE} ("Dice")) -> ()
              }
              event "Dice": Value Change {
                n171 = event-data() -> ()  [unwired: 1 in, 6 out]
                n172 = local write "Dice"(cluster{"Boolean 2":bool, "Dice":bool} {"Boolean 2"=TRUE, "Dice"=FALSE} ("Dice")) -> ()
              }
              event "CapitalOnly", "Font Compression": Value Change {
                n173 = event-data() -> ()  [unwired: 1 in, 1 out]
              }
              event Mouse Enter; Mouse Leave {
                n174 = event-data() -> ("Type"=w375:T12, "CtlRef"=w379:refnum<vi>)  [unwired: 1 in]
                n175 = Equal?(x=w375, y=lveventtype."Mouse Enter") -> (x = y?=w373:bool)
                n176 = property class="Clust (strict)"(reference=w379) -> (reference out=w378:refnum<vi>, "Value"=w377:T13)  [unwired: 1 in, 1 out]
                n177 = Bundle By Name(cluster=w377, "Decal"=w373) -> (w376:T13)
                n178 = property class="Clust (strict)"(reference=w378, "Value"=w376) -> ()  [unwired: 1 in, 2 out]
              }
              event "Rows": Value Change {
                n179 = event-data() -> ()  [unwired: 1 in, 1 out]
                n180 = case shown="\"1 Row\", Default" "Rows" {
                  tunnel: [u8 7 ("Icon Header Size") u8 13 ("Icon Header Size") u8 19 ("Icon Header Size")] -> w382
                  frame "1 Row", Default {
                  }
                  frame "2 Rows" {
                  }
                  frame "3 Rows" {
                  }
                }
                n181 = local write "Height (pixels)"(w382) -> ()
              }
              event "Thickness (pixels)": Value Change {
                (unwired) "UpdateIcons"
                n182 = event-data() -> ()  [unwired: 1 in, 1 out]
              }
              event "Height (pixels)": Value Change {
                (unwired) "UpdateIcons"
                n183 = event-data() -> ()  [unwired: 1 in, 1 out]
                n184 = Quotient & Remainder(x="Height (pixels)", y=u8 5) -> (floor(x/y)=w391:u8)  [unwired: 1 out]
                n185 = case shown="3.." w391 {
                  tunnel: [enum16{"1 Row", "2 Rows", "3 Rows"}."1 Row" ("Rows") enum16{"1 Row", "2 Rows", "3 Rows"}."2 Rows" ("Rows") enum16{"1 Row", "2 Rows", "3 Rows"}."3 Rows" ("Rows")] -> w392
                  frame 1, Default {
                  }
                  frame 2 {
                  }
                  frame 3.. {
                  }
                }
                n186 = local write "Rows"(w392) -> ()
              }
              event "OK": Value Change {
                n187 = event-data() -> ()  [unwired: 1 in, 6 out]
              }
              event "_LastHeaders": Mouse Down {
                n188 = event-data() -> ("Button"=w400:u16, "Coords"=w404:T1)  [unwired: 1 in]
                n189 = case shown="1" w400 {
                  tunnel: w404 -> [_ w424]
                  tunnel: ["Idle" w423] -> w403
                  tunnel: [w406 w422] -> w402
                  tunnel: w401 -> [w406 w416]
                  frame 0, Default {
                  }
                  frame 1 {
                    n190 = property on="_LastHeaders" class="Arr (strict)" props=["MasterRect", "Index Values", "Top"]() -> ("MasterRect"=w409:T14, "Index Values"=w417:u32[])  [unwired: 2 in, 3 out]
                    n191 = Unbundle By Name(w424) -> ("Vertical"=w421:i32)
                    n192 = Unbundle By Name(w416) -> ("Headers"=w415:cluster{"Header":u8[][]}[])
                    n193 = Unbundle By Name(w409) -> ("Top"=w408:i16)
                    n194 = Subtract(x=w421, y=w408) -> (x-y=w420:i32)
                    n195 = Index Array(array=w417) -> (element=w413:u32)  [unwired: 1 in]
                    n196 = Divide(x=w420, y=65) -> (x/y=w418:dbl)
                    n197 = Round Toward -Infinity(1:w418) -> (0:w407:dbl)
                    n198 = Add(x=w413, y=w407) -> (x+y=w414:dbl)
                    n199 = Index Array(array=w415, index=w414) -> (element=w412:cluster{"Header":u8[][]})
                    n200 = Unbundle By Name(w412) -> ("Header"=w411:u8[][])
                    n201 = Empty Array?(array=w411) -> (empty?=w410:bool)
                    n202 = case shown="False" w410 {
                      tunnel: ["HeaderOCR" "Idle"] -> w423
                      tunnel: [w430 w436] -> w422
                      tunnel: w416 -> [w429 w436]
                      tunnel: w411 -> [w428 _]
                      frame False {
                        n203 = Array Size(array=w428) -> (size(s)=w427:i32[])
                        n204 = Bundle By Name(cluster=w429, "Header"=w428) -> (w430:T6)
                        n205 = Index Array(array=w427) -> (element=w426:i32)  [unwired: 1 in]
                        n206 = case shown="17.., Default" w426 {
                          tunnel: [enum16{"1 Row", "2 Rows", "3 Rows"}."1 Row" ("Rows") enum16{"1 Row", "2 Rows", "3 Rows"}."2 Rows" ("Rows") enum16{"1 Row", "2 Rows", "3 Rows"}."3 Rows" ("Rows")] -> w425
                          frame ..10 {
                          }
                          frame 11..16 {
                          }
                          frame 17.., Default {
                          }
                        }
                        n207 = local write "Rows"(w425) -> ()
                        n208 = local write "Height (pixels)"(w426) -> ()
                      }
                      frame True {
                      }
                    }
                    "Coords" <- w424
                  }
                }
              }
              event "_LastHeaders": Shortcut Menu Selection (User) {
                n209 = event-data() -> ("Coords"=w443:T1)  [unwired: 1 in, 2 out]
                "Coords 2" <- w443
                n210 = property on="_LastHeaders" class="Arr (strict)" props=["MasterRect", "Index Values", "Top"]() -> ("MasterRect"=w446:T14, "Index Values"=w449:u32[])  [unwired: 2 in, 3 out]
                n211 = Unbundle By Name(w443) -> ("Vertical"=w453:i32)
                n212 = Unbundle By Name(w446) -> ("Top"=w445:i16)
                n213 = Unbundle By Name(w441) -> ("Headers"=w448:cluster{"Header":u8[][]}[], "Names"=w442:string[])
                n214 = Subtract(x=w453, y=w445) -> (x-y=w452:i32)
                n215 = Index Array(array=w449) -> (element=w447:u32)  [unwired: 1 in]
                n216 = Divide(x=w452, y=65) -> (x/y=w450:dbl)
                n217 = Round Toward -Infinity(1:w450) -> (0:w444:dbl)
                n218 = Add(x=w447, y=w444) -> (x+y=w437:dbl)
                n219 = Delete From Array(array=w448, index=w437) -> (array with subset deleted=w438:cluster{"Header":u8[][]}[])  [unwired: 1 in, 1 out]
                n220 = Delete From Array(array=w442, index=w437) -> (array with subset deleted=w439:string[])  [unwired: 1 in, 1 out]
                n221 = Bundle By Name(cluster=w441, "Headers"=w438, "Names"=w439) -> (w440:T6)
              }
              event "Cancel": Value Change {
                n222 = event-data() -> ()  [unwired: 1 in, 6 out]
                n223 = Bundle By Name(cluster=w456, "Cancel"=TRUE) -> (w455:T6)
              }
            }
          }
          frame "HeaderOCR" {
            w482 = 0 ("index (row)")
            w487 = u8 255  # Black(8bit)
            n224 = Unbundle By Name(w494) -> ("Header"=w460:u8[][])
            n225 = Array Size(array=w460) -> (size(s)=w485:i32[])
            n226 = Index Array(array=w485) -> (element #1=w484:i32, element #2=w483:i32)  [unwired: 2 in]
            n227 = Array Size(array=w460) -> (size(s)=w493:i32[])
            n228 = Decrement(x=w484) -> (x-1=w481:i32)
            n229 = Decrement(x=w483) -> (x-1=w480:i32)
            n230 = Multiply Array Elements(1:w493) -> (0:w491:i32)
            n231 = Index Array(array=w460) -> (element=w475:u8[])  [unwired: 2 in]
            n232 = Reshape Array(w460, w491) -> (w492:u8[])
            n233 = Index Array(array=w460, index (row) #1=0 ("index (row)"), index (col) #1=4 ("disabled index (col)"), index (row) #2=w482, index (col) #2=w482, index (row) #3=w482, index (col) #3=w480, index (row) #4=w481, index (col) #4=w482, index (row) #5=w481, index (col) #5=w480) -> (element #1=w468:u8, element #2=w479:u8, element #3=w478:u8, element #4=w477:u8, element #5=w476:u8)
            n234 = Decrement(x=w491) -> (x-1=w490:i32)
            n235 = Array Max & Min(array=w475) -> (max value=w472:u8, min value=w474:u8)  [unwired: 2 out]
            n236 = Equal?(x=w472, y=w474) -> (x = y?=w473:bool)
            n237 = Build Array(w468, w479, w478, w477, w476) -> (w467:u8[])
            n238 = for {
              tunnel: w467 -> [w499] mode=indexing
              shift-right: [w497] -> w465
              shift-left: u8[] [] -> [w498]
              n239 = case shown="255" w499 {
                selector: w499 -> [w500 _]
                tunnel: w498 -> [w502 w503]
                tunnel: [w501 w503] -> w497
                frame Default {
                  n240 = Build Array (concatenate)(w502, w500) -> (w501:u8[])
                }
                frame 255 {
                }
              }
            }
            n241 = call <vilib>:"Median.vi"("X"=w465) -> ("median"=w471:dbl)  [unwired: 1 out]
            n242 = To Unsigned Byte Integer(number=w471) -> (unsigned 8bit integer=w464:u8)
            n243 = Select(t=w472, s=w473, f=w464) -> (s? t:f=w459:u8)
            n244 = for {
              tunnel: w492 -> [w505] mode=indexing
              tunnel: w459 -> [w506]
              tunnel: w490 -> [_]
              tunnel: [w504] -> w489
              tunnel: [w505] -> w488
              stop <- w504 stop-if-true
              n245 = Not Equal?(x=w506, y=w505) -> (x != y?=w504:bool)
            }
            n246 = Select(t=w488, s=w489, f=w487) -> (s? t:f=w486:u8)
            n247 = Build Array(w486, w459) -> (w496:u8[])
            n248 = for {
              tunnel: [w509] -> w461
              tunnel: w460 -> [w511]
              tunnel: bool[] [FALSE, TRUE] -> [w510] mode=indexing
              tunnel: w496 -> [w507] mode=indexing
              stop <- w508 continue-if-true
              n249 = call <resource>:"GOOP_IconOCR.vi"("BackColor(T), TextColor(F)"=w510, "BackColor Or TextColor(8bit)"=w507, "Icon"=w511) -> ("String"=w509:string)  [unwired: 8 in]
              n250 = Empty String/Path?(string/path=w509) -> (empty?=w508:bool)
            }
            n251 = local write "Text"(w461) -> ()
          }
          frame "RandomColors" {
            w518 = T3 {"Decal"=FALSE, "Color"=0} ("Public")
            w521 = u32[] [15007601, 14876576, 16751729, 15400704, 15507711, 16775072, 12713864, 12124142, 16776704, 16754080, 16752888, 16383904, 7667498, 16754986, 12112639, 3079936, 16776704, 16745561, 9341183, 16746660, 16773906, 2792191, 16762993, 5766954, 16318226, 15517125, 13290186, 10197915, 7442943, 11316396, 9743236, 16757617, 16767648, 6618880, 16711680, 16860, 16860, 16773906, 65421, 2789375, 13714175, 12827549, 10595204, 7641720, 6062466, 8025242, 11507131, 10386594, 786176, 8584960, 16318208, 16731648, 16755616, 16734715, 14399157, 16754801, 16714752, 10026888, 3524608]
            n252 = Random Number (0-1)() -> (number: 0 to 1=w532:dbl)
            n253 = Random Number (0-1)() -> (number: 0 to 1=w524:dbl)
            n254 = Array Size(array=w521) -> (size(s)=w523:i32)
            n255 = Build Array (concatenate)(w521, u32[] [10427904, 10442496, 10444544, 10452224, 10458112, 5927680, 3633920, 1351424, 35084, 40813, 16959, 19615, 1376393, 4194441, 10748084, 10420349, 7536704, 8978459, 5963776, 3882593, 4944486, 5204291, 7553536, 5263440, 4013373, 2763306, 6447714, 9540204, 6982244, 5470832, 6056066, 40848, 11010228]) -> (w530:u32[])
            n256 = Array Size(array=w530) -> (size(s)=w533:i32)
            n257 = Multiply(x=w523, y=w524) -> (x*y=w525:dbl)
            n258 = Multiply(x=w533, y=w532) -> (x*y=w531:dbl)
            n259 = Round Toward -Infinity(1:w525) -> (0:w522:dbl)
            n260 = Round Toward -Infinity(1:w531) -> (0:w529:dbl)
            n261 = Index Array(array=w521, index=w522) -> (element=w515:u32)
            n262 = Index Array(array=w530, index=w529) -> (element=w517:u32)
            n263 = Greater?(x=w529, y=w523) -> (0:w528:bool)
            n264 = Select(t=u32 16777215, s=w528, f=u32 0) -> (s? t:f=w516:u32)
            n265 = Bundle By Name(cluster=w518, "Color"=u32 0) -> ()  [unwired: 1 out]
            n266 = Bundle By Name(cluster=w518, "Color"=w517) -> (w514:T3)
            n267 = Bundle By Name(cluster=w518, "Color"=w516) -> (w513:T3)
            n268 = Bundle By Name(cluster=w518, "Color"=w515) -> ()  [unwired: 1 out]
            n269 = local write "HeaderBk"(w514) -> ()
            n270 = local write "HeaderText"(w513) -> ()
          }
          frame "UpdateLastHeaders" {
            n271 = Unbundle By Name(w545) -> ("Header"=w536:u8[][], "Headers"=w542:cluster{"Header":u8[][]}[], "Names"=w541:string[])
            n272 = for {
              tunnel: w542 -> [w579] mode=indexing
              tunnel: w536 -> [w577]
              tunnel: [w576] -> w544
              tunnel: [w575] -> w543
              i -> [w575]
              stop <- w576 stop-if-true
              n273 = Unbundle By Name(w579) -> ("Header"=w578:u8[][])
              n274 = Equal?(x=w577, y=w578) -> (x = y?=w576:bool)
            }
            n275 = case shown="False" w544 {
              tunnel: w543 -> [_ w561]
              tunnel: w542 -> [w552 w560]
              tunnel: w541 -> [w550 w559]
              tunnel: w540 -> [w549 w558]
              tunnel: w539 -> [w548 w557]
              tunnel: w536 -> [w547 _]
              frame False {
                n276 = Bundle("Header"=w547) -> (w546:cluster{"Header":u8[][]})  [unwired: 1 in]
                n277 = local read "Text"() -> (w551:string)
                n278 = Build Array (concatenate)(w551, w550) -> (w556:string[])
                n279 = Build Array (concatenate)(w546, w552) -> (w555:cluster{"Header":u8[][]}[])
                n280 = Bundle By Name(cluster=w549, "Headers"=w555, "Names"=w556) -> (w554:T4)
                n281 = Flatten To String(anything=w554) -> (data string=w553:string)  [unwired: 3 in, 2 out]
                n282 = Write to Text File(file (use dialog)=w548, text=w553) -> ()  [unwired: 2 in, 3 out]
              }
              frame True {
                n283 = case shown="Default" w561 {
                  selector: w561 -> [_ w570]
                  tunnel: w560 -> [_ w574]
                  tunnel: w559 -> [_ w571]
                  tunnel: w558 -> [_ w567]
                  tunnel: w557 -> [_ w562]
                  frame 0 {
                  }
                  frame Default {
                    n284 = Delete From Array(array=w571, index=w570) -> (array with subset deleted=w569:string[])  [unwired: 1 in, 1 out]
                    n285 = Delete From Array(array=w574, index=w570) -> (deleted portion=w573:cluster{"Header":u8[][]}, array with subset deleted=w572:cluster{"Header":u8[][]}[])  [unwired: 1 in]
                    n286 = local read "Text"() -> (w568:string)
                    n287 = Build Array (concatenate)(w568, w569) -> (w566:string[])
                    n288 = Build Array (concatenate)(w573, w572) -> (w565:cluster{"Header":u8[][]}[])
                    n289 = Bundle By Name(cluster=w567, "Headers"=w565, "Names"=w566) -> (w564:T4)
                    n290 = Flatten To String(anything=w564) -> (data string=w563:string)  [unwired: 3 in, 2 out]
                    n291 = Write to Text File(file (use dialog)=w562, text=w563) -> ()  [unwired: 2 in, 3 out]
                  }
                }
              }
            }
          }
        }
        n292 = Equal?(x=w54, y="Exit") -> (x = y?=w57:bool)
        n293 = Select(t="Error", s=w53, f=w54) -> (s? t:f=w58:string)
      }
    }
    frame Error {
    }
  }
  "error out" <- w13
  n294 = stacked-sequence {
    tunnel: w13 -> [_]
    tunnel: [w584] -> w12
    tunnel: [w582] -> w11
    tunnel: [w581] -> w1
    frame #0 {
      n295 = local read "Thickness (pixels)"() -> (w584:u8)
      n296 = local read "Frame"() -> (w583:T3)
      n297 = local read "NoSplitter"() -> (w581:bool)
      n298 = Unbundle By Name(w583) -> ("Color"=w582:u32)
    }
  }
  "FrameColorOut" <- w11
  "FrameThicknessOut" <- w12
  "NoSplitterOut" <- w1
  n299 = Unbundle By Name(w16) -> ("Cancel"=→"Cancelled":bool, "Header"=→"HeaderIconOut":u8[][])  [unwired: 1 out]
